vi "Prepare Build Specification.vi"(6 "Cleared Compiled Object Cache":bool, 8 "error in":errorcluster, 9 "Set PPL Version":bool, 10 "Build Specification Version":T1, 11 "Runner in":refnum<class "Runner.lvclass">) -> (0 "error out":errorcluster, 3 "Runner out":refnum<class "Runner.lvclass">)   [LabVIEW 2026, in "Runner.lvlib" / "Runner.lvclass"]
doc: "Prepare build specification for building process."
uses:
  Runner.lvclass
  <vilib>/AppBuilder/AB_API_Simple/Build Specification Version.ctl
  Runner.lvclass/Runner.ctl
  Interfaces/ILogger/ILogger Messages/Log Msg/Log Msg.lvclass/Log Msg.ctl
  <vilib>/ActorFramework/Message Enqueuer/Message Enqueuer.lvclass/Message Enqueuer.ctl
  <vilib>/ActorFramework/Message Enqueuer/Enqueue.vi
  Interfaces/ILogger/ILogger Messages/Log Msg/Log Msg.lvclass
  C:/Program Files/National Instruments/LabVIEW 2026/vi.lib/ActorFramework/Message/Message.lvclass
  <userlib>/_OpenG.lib/file/file.llb/Strip Path Extension - String__ogtk.vi
  <vilib>/ActorFramework/Message Priority Queue/Priority Enqueue.vi
  Interfaces/IFile Manager/IFile Manager.lvclass
  Interfaces/IProject Manager/IProject Manager.lvclass
  <userlib>/_OpenG.lib/file/file.llb/openg_file.lvlib
  <vilib>/AppBuilder/AB_API_Simple/NI_App_Builder_API.lvlib
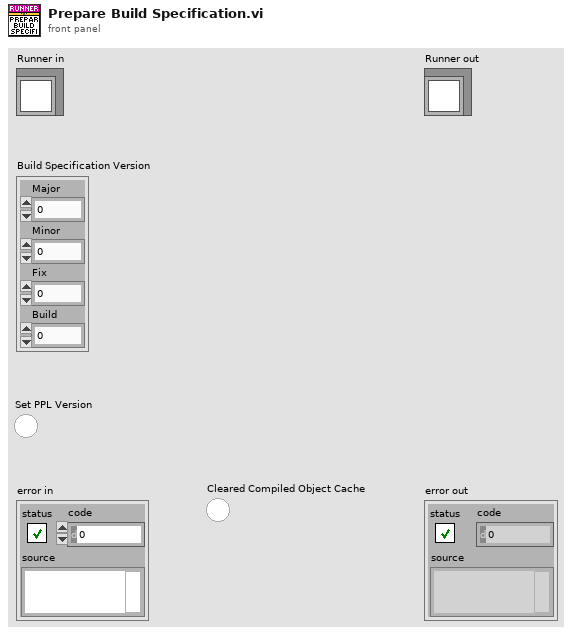
[diagram p1: front panel]
types:
  T1 = typedef "NI_App_Builder_API.lvlib/Build Specification Version.ctl" = cluster{"Major":u16, "Minor":u16, "Fix":u16, "Build":u16}
  T2 = typedef "Log Entry--cluster.ctl" = cluster{"Time":timestamp, "Message":string}
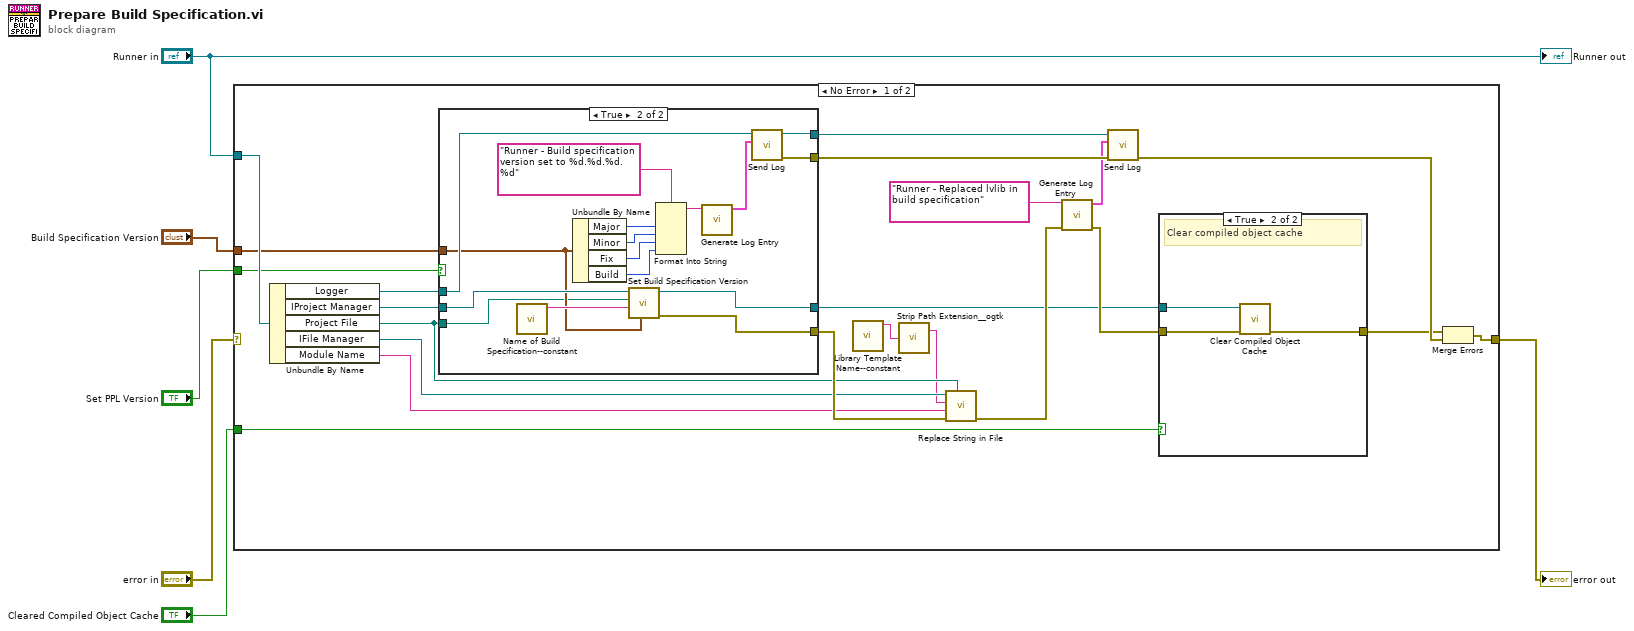
[diagram p0: block diagram]
diagram:
  n1 = case shown="No Error" "error in" {
    selector: "error in" -> [_ w51]
    tunnel: "Runner in" -> [w21 _]
    tunnel: "Build Specification Version" -> [w15 _]
    tunnel: [w27 w51] -> w5
    tunnel: "Set PPL Version" -> [w9 _]
    tunnel: "Cleared Compiled Object Cache" -> [w8 _]
    frame No Error {
      n2 = Unbundle By Name(w21) -> ("Logger"=w19:refnum<class "Message Enqueuer.lvclass">, "IProject Manager"=w20:refnum<class "IProject Manager.lvclass">, "Project File"=w12:path, "IFile Manager"=w14:refnum<class "IFile Manager.lvclass">, "Module Name"=w13:string)
      n3 = case shown="True" w9 {
        tunnel: [_ w50] -> w28
        tunnel: w20 -> [w33 w48]
        tunnel: w19 -> [w34 w41]
        tunnel: [w34 w39] -> w17
        tunnel: w15 -> [_ w37]
        tunnel: [_ w49] -> w26
        tunnel: w12 -> [_ w36]
        tunnel: [w33 w35] -> w7
        frame False {
        }
        frame True {
          n4 = call "Name of Build Specification--constant.vi"() -> ("Name of Build Specification"=w38:string)  [unwired: 11 in]
          n5 = Unbundle By Name(w37) -> ("Major"=w46:u16, "Minor"=w45:u16, "Fix"=w44:u16, "Build"=w43:u16)
          n6 = call-dynamic "Set Build Specification Version.vi"("Build Specification Version"=w37, "Build Specification"=w38, "Project File"=w36, "IProject Manager in"=w48) -> ("error out"=w49:errorcluster, "IProject Manager out"=w35:refnum<class "IProject Manager.lvclass">)  [unwired: 6 in]
          n7 = Format Into String(format string="Runner - Build specification version set to %d.%d.%d.%d", w46, w45, w44, w43) -> (resulting string=w42:string)  [unwired: 2 in, 1 out]
          n8 = call "Generate Log Entry.vi"("Message"=w42) -> ("Log Entry"=w40:T2)  [unwired: 9 in, 1 out]
          n9 = call "Send Log.vi"("Log Entry"=w40, "Message Enqueuer"=w41) -> ("error out"=w50:errorcluster, "Message Enqueuer out"=w39:refnum<class "Message Enqueuer.lvclass">)  [unwired: 8 in]
        }
      }
      n10 = call "Library Template Name--constant.vi"() -> ("Library Template Name"=w11:string)  [unwired: 11 in]
      n11 = call-poly <userlib>:"Strip Path Extension__ogtk.vi"("path"=w11) -> ("root"=w10:string)  [unwired: 1 out]
      n12 = call-dynamic "Replace String in File.vi"("File Path"=w12, "error in"=w26, "Replace String"=w13, "Search String"=w10, "IFile Manager in"=w14) -> ("error out"=w25:errorcluster)  [unwired: 5 in, 1 out]
      n13 = call "Generate Log Entry.vi"("error in"=w25, "Message"="Runner - Replaced lvlib in build specification") -> ("error out"=w24:errorcluster, "Log Entry"=w16:T2)  [unwired: 8 in]
      n14 = call "Send Log.vi"("error in (no error)"=w28, "Log Entry"=w16, "Message Enqueuer"=w17) -> ("error out"=w23:errorcluster)  [unwired: 7 in, 1 out]
      n15 = case shown="True" w8 {
        tunnel: w7 -> [_ w30]
        tunnel: w24 -> [w29 w32]
        tunnel: [w29 w31] -> w22
        frame False {
          # "No action"
        }
        frame True {
          # "Clear compiled object cache"
          n16 = call-dynamic "Clear Compiled Object Cache.vi"("error in"=w32, "IProject Manager in"=w30) -> ("error out"=w31:errorcluster)  [unwired: 8 in, 1 out]
        }
      }
      n17 = Merge Errors(w22, w23) -> (w27:errorcluster)
    }
    frame Error {
      # "Pass error without further action."
    }
  }
  "error out" <- w5
  "Runner out" <- "Runner in"
